vi "HP Loop.vi"(8 "error in (no error)":errorcluster, 11 "ValveControlModule in":refnum<class "DigitalControlModule.lvclass">) -> (0 "error out":errorcluster, 3 "ValveControlModule out":refnum<class "DigitalControlModule.lvclass">)   [LabVIEW 2023, in "VolatusControl.lvlib" / "DigitalControlModule.lvclass"]
uses:
  DigitalControlModule.lvclass
  DigitalControlModule.lvclass/DigitalControlModule.ctl
  <vilib>/Platform/TimedLoop/XDataNode/timing_clust.ctl
  <vilib>/Platform/TimedLoop/XDataNode/nitl_modes.ctl
  <vilib>/Platform/TimedLoop/XDataNode/wakeup.ctl
  Volatus/Module/Module.lvclass
  Volatus/Module/Module.lvclass/Module.ctl
  messages/CmdDigital/Class/Msg.lvclass
  messages/CmdDigital/Class/Msg.lvclass/Msg.ctl
  Volatus/MessageQ/MessageQ.lvclass/MessageQ.ctl
  messages/CmdDigital/Data.ctl
  messages/CmdDigitalMultiple/Data.ctl
  messages/CmdAnalog/Class/Msg.lvclass
  messages/CmdAnalog/Class/Msg.lvclass/Msg.ctl
  messages/CmdAnalog/Data.ctl
  Volatus/Module/Self Q.vi
  Volatus/MessageQ/Send.vi
  Volatus/Module/Report Event.vi
  lv-vecto/Vecto/Bool to String.vi
  lv-vecto/Vecto/Group DBL/Group DBL.lvclass
  <vilib>/Utility/error.llb/Error Cluster From Error Code.vi
  Volatus/VolatusAPI/Report Event.vi
  <vilib>/platform/TimedLoop/XDataNode/XDataNode.xnode
  <vilib>/Platform/TimedLoop/XDataNode/XDNodeRunTimeDep.lvlib
  messages/CmdDigital/CmdDigital.lvlib
  messages/CmdDigitalMultiple/CmdDigitalMultiple.lvlib
  messages/CmdAnalog/CmdAnalog.lvlib
  lv-vecto/Vecto/Group/Group.lvclass
  C:/dev/volatus/mts-volatus-super/libs/lv-volatus/Volatus/Module/Module.lvclass
  C:/dev/volatus/mts-volatus-super/libs/lv-volatus/VolatusControl/DigitalControlModule/DigitalControlModule.lvclass
  messages/CmdDigitalMultiple/Class/Msg.lvclass
  C:/dev/volatus/mts-volatus-super/libs/lv-volatus/messages/CmdDigital/Class/Msg.lvclass
  C:/dev/volatus/mts-volatus-super/libs/lv-protoc/LV-Proto/Message/Message.lvclass
  C:/dev/volatus/mts-volatus-super/libs/lv-volatus/messages/CmdDigitalMultiple/Class/Msg.lvclass
  C:/dev/volatus/mts-volatus-super/libs/lv-volatus/messages/CmdAnalog/Class/Msg.lvclass
  C:/dev/volatus/mts-volatus-super/libs/lv-vecto/Vecto/Group/Group.lvclass
  C:/dev/volatus/mts-volatus-super/libs/lv-vecto/Vecto/Group DBL/Group DBL.lvclass
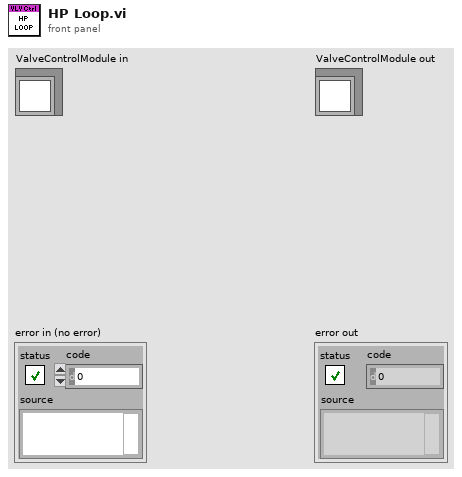
[diagram p1: front panel]
types:
  T1 = typedef "XDNodeRunTimeDep.lvlib/timing_clust.ctl" = cluster{"Expected End [f-1]":u64, "Actual End [f-1]":u64, "Finished Late? [f-1]":bool, "Expected End [i-1]":u64, "Actual End [i-1]":u64, "Finished Late? [i-1]":bool, "Expected Start [i]":u64, "Actual Start [i]":u64, "Expected Start [f]":u64, "Actual Start [f]":u64, "Source Name":string, "Structure Name":string, "Period":i64, "Deadline":i64, "Offset":i64, "Start":i64, "Priority":i32, "Timeout":i32, "Mode":T2, "Wakeup Reason":T3, "Error":errorcluster, "Source Type":string, "Secondary Source Type":string, "Global End Time":u64, "Global Start Time":u64, "Frame Duration":u64, "Iteration Duration":u64, "Assigned CPU":i32, "I/O Scan Engine Mode":u32}
  T2 = typedef "XDNodeRunTimeDep.lvlib/nitl_modes.ctl" = enum32{"No Change", "Process missed periods, maintain original phase", "Discard missed periods, maintain original phase", "Process missed periods, ignore original phase", "Discard missed periods, ignore original phase"}
  T3 = typedef "XDNodeRunTimeDep.lvlib/wakeup.ctl" = enum32{"Normal", "Aborted", "Asynchronous wakeup", "Timing source error", "Timed loop error", "Timeout"}
  T4 = enum32{"Invalid", "Standard", "Closed", "Hidden", "Minimized", "Maximized"}
  T5 = typedef "CmdDigital.lvlib/Data.ctl" = cluster{"channel":string, "value":bool}
  T6 = typedef "CmdDigitalMultiple.lvlib/Data.ctl" = cluster{"values":T5[]}
  T7 = typedef "CmdAnalog.lvlib/Data.ctl" = cluster{"channel":string, "value":dbl}
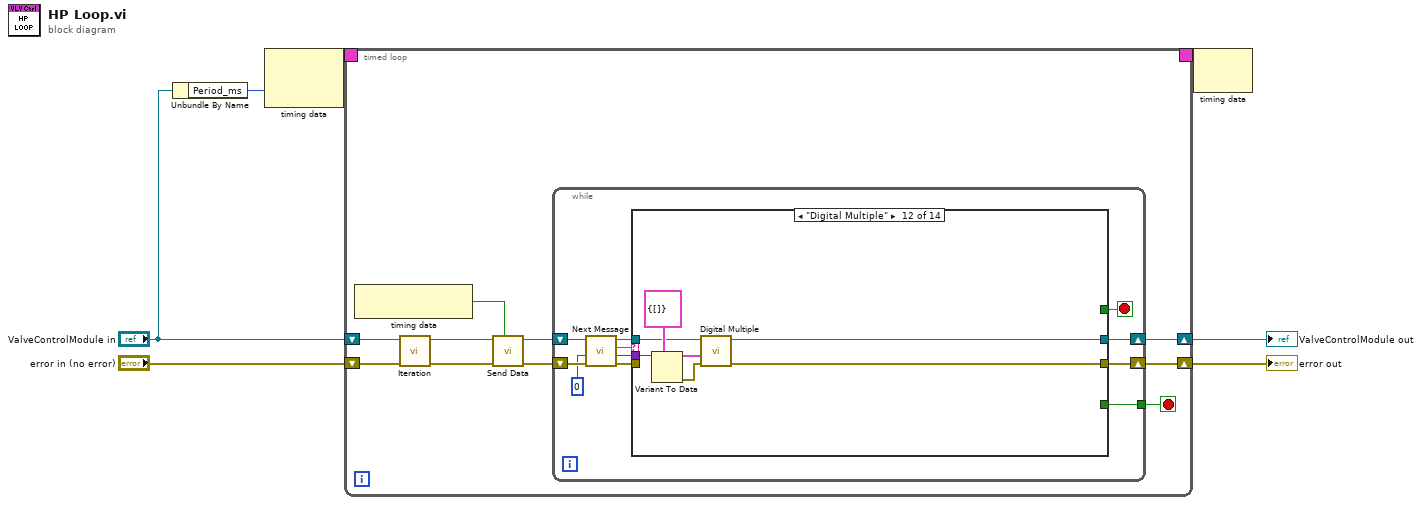
[diagram p0: block diagram]
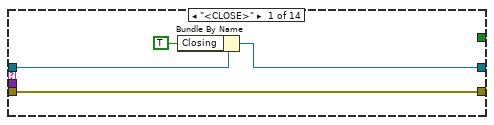
[diagram p2: hidden frame]
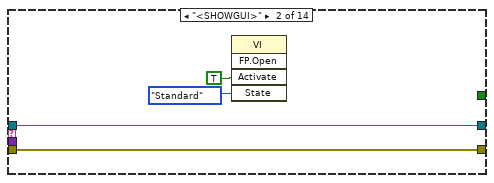
[diagram p3: hidden frame]
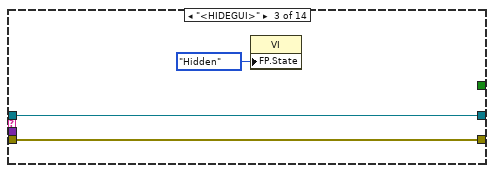
[diagram p4: hidden frame]
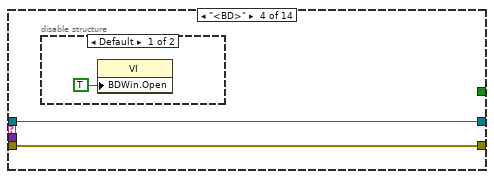
[diagram p5: hidden frame]
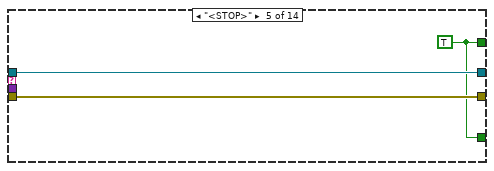
[diagram p7: hidden frame]
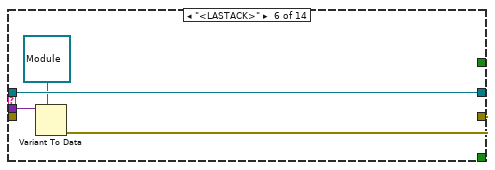
[diagram p8: hidden frame]
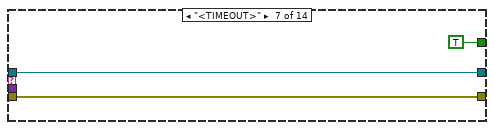
[diagram p9: hidden frame]
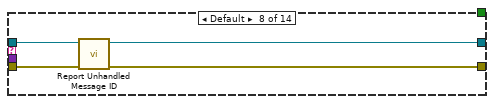
[diagram p10: hidden frame]
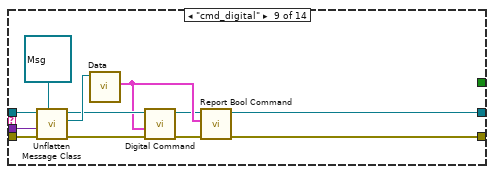
[diagram p11: hidden frame]
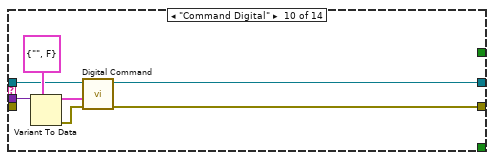
[diagram p12: hidden frame]
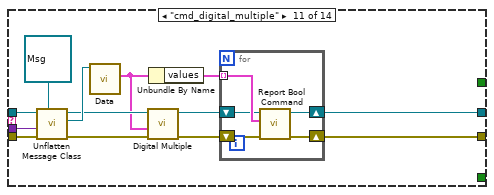
[diagram p13: hidden frame]
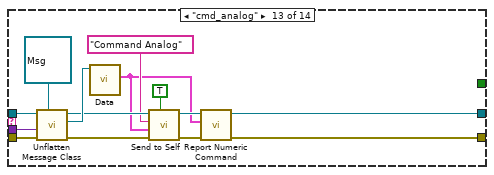
[diagram p14: hidden frame]
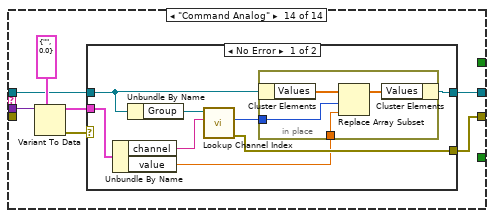
[diagram p15: hidden frame]
diagram:
  n1 = Unbundle By Name("ValveControlModule in") -> ("Period_ms"=w1:i64)
  n2 = node-c288(w1) -> (w7:T1)  [unwired: 1 in]
  n3 = timed-loop {
    shift-right: [w17] -> w4
    shift-left: "ValveControlModule in" -> [w12]
    shift-right: [w16] -> w3
    shift-left: "error in (no error)" -> [w11]
    timing: w7 -> [_]
    timing-out: [_] -> w6
    stop <- w15 stop-if-true
    n4 = node-c288() -> (w8:bool)  [unwired: 1 in]
    n5 = call "Iteration.vi"("error in (no error)"=w11, "ValveControlModule in"=w12) -> ("error out"=w13:errorcluster, "ValveControlModule out"=w14:refnum<class "DigitalControlModule.lvclass">)  [unwired: 8 in]
    n6 = call "Send Data.vi"("Finished Late"=w8, "error in (no error)"=w13, "ValveControlModule in"=w14) -> ("error out"=w10:errorcluster, "ValveControlModule out"=w9:refnum<class "DigitalControlModule.lvclass">)  [unwired: 7 in]
    n7 = while {
      tunnel: [w25] -> w15
      shift-right: [w26] -> w16
      shift-left: w10 -> [w23]
      shift-right: [w27] -> w17
      shift-left: w9 -> [w22]
      stop <- w20 stop-if-true
      n8 = call "Next Message.vi"("error in (no error)"=w23, "Timeout ms (-1)"=0, "Module in"=w22) -> ("error out"=w30:errorcluster, "Data"=w24:variant, "ID"=w29:string, "Module out"=w28:refnum<class "DigitalControlModule.lvclass">)  [unwired: 5 in]
      n9 = case shown="\"Digital Multiple\"" w29 {
        tunnel: w30 -> [w34 w37 w40 w42 w46 _ w53 w58 w69 _ w89 _ w115 _]
        tunnel: w28 -> [w33 w38 w41 w43 w47 w51 w54 w56 w70 w75 w90 w100 w116 w119]
        tunnel: [w32 w38 w41 w43 w47 w51 w54 w55 w64 w72 w84 w97 w104 w117] -> w27
        tunnel: [w34 w37 w40 w42 w46 w48 w53 w57 w65 w73 w85 w98 w106 w118] -> w26
        tunnel: [_ _ _ _ w45 _ _ _ _ _ _ _ _ _] -> w25
        tunnel: w24 -> [_ _ _ _ _ w50 _ _ w68 w77 w88 w102 w114 w123]
        tunnel: [_ _ _ _ w45 _ TRUE _ _ _ _ _ _ _] -> w20
        frame "<CLOSE>" {
          n10 = Bundle By Name(cluster=w33, "Closing"=TRUE) -> (w32:refnum<class "DigitalControlModule.lvclass">)
        }
        frame "<SHOWGUI>" {
          n11 = invoke class="VI" method="FP.Open"("Activate"=TRUE ("Activate?"), "State"=T4."Standard") -> ()  [unwired: 3 in, 5 out]
        }
        frame "<HIDEGUI>" {
          n12 = property class="VI"("FP.State"=T4."Hidden" ("Front Panel Window:State")) -> ()  [unwired: 2 in, 2 out]
        }
        frame "<BD>" {
          n13 = disable-structure shown="Default" {
            frame condition #0 (active) {
              n14 = property class="VI"("BDWin.Open"=TRUE ("Block Diagram Window:Open")) -> ()  [unwired: 2 in, 2 out]
            }
            frame condition #1 {
            }
          }
        }
        frame "<STOP>" {
          w45 = TRUE
        }
        frame "<LASTACK>" {
          n15 = Variant To Data(type=refnum<class "Module.lvclass"> refnum ("Volatus:Module"), Variant=w50) -> (error out=w48:errorcluster)  [unwired: 1 in, 1 out]
        }
        frame "<TIMEOUT>" {
        }
        frame Default {
          n16 = call "Report Unhandled Message ID.vi"("error in (no error)"=w58, "Module in"=w56) -> ("error out"=w57:errorcluster, "Module out"=w55:refnum<class "DigitalControlModule.lvclass">)  [unwired: 8 in]
        }
        frame "cmd_digital" {
          n17 = call "Unflatten Message Class.vi"("Message Type"=refnum<class "Msg.lvclass"> refnum ("CmdDigital.lvlib:Msg.lvclass"), "error in (no error)"=w69, "Data"=w68, "Module in"=w70) -> ("error out"=w62:errorcluster, "Message"=w66:refnum<class "Msg.lvclass">, "Module out"=w63:refnum<class "DigitalControlModule.lvclass">)  [unwired: 4 in, 1 out]
          n18 = call "Data.vi"("PB Msg Template in"=w66) -> ("Data"=w61:T5)  [unwired: 8 in, 2 out]
          n19 = call "Digital Command.vi"("error in (no error)"=w62, "CmdDigital"=w61, "ValveControlModule in"=w63) -> ("error out"=w59:errorcluster, "ValveControlModule out"=w60:refnum<class "DigitalControlModule.lvclass">)  [unwired: 7 in]
          n20 = call "Report Bool Command.vi"("error in (no error)"=w59, "Command"=w61, "Module in"=w60) -> ("error out"=w65:errorcluster, "Module out"=w64:refnum<class "DigitalControlModule.lvclass">)  [unwired: 7 in]
        }
        frame "Command Digital" {
          n21 = Variant To Data(type=T5 {"channel"="", "value"=FALSE} ("CmdDigital"), Variant=w77) -> (data=w71:T5, error out=w74:errorcluster)  [unwired: 1 in]
          n22 = call "Digital Command.vi"("error in (no error)"=w74, "CmdDigital"=w71, "ValveControlModule in"=w75) -> ("error out"=w73:errorcluster, "ValveControlModule out"=w72:refnum<class "DigitalControlModule.lvclass">)  [unwired: 7 in]
        }
        frame "cmd_digital_multiple" {
          n23 = call "Unflatten Message Class.vi"("Message Type"=refnum<class "Msg.lvclass"> refnum ("CmdDigitalMultiple.lvlib:Msg.lvclass"), "error in (no error)"=w89, "Data"=w88, "Module in"=w90) -> ("error out"=w82:errorcluster, "Message"=w86:refnum<class "Msg.lvclass">, "Module out"=w83:refnum<class "DigitalControlModule.lvclass">)  [unwired: 4 in, 1 out]
          n24 = call "Data.vi"("PB Msg Template in"=w86) -> ("Data"=w81:T6)  [unwired: 8 in, 2 out]
          n25 = call "Digital Multiple.vi"("error in (no error)"=w82, "Data"=w81, "ValveControlModule in"=w83) -> ("error out"=w78:errorcluster, "ValveControlModule out"=w79:refnum<class "DigitalControlModule.lvclass">)  [unwired: 7 in]
          n26 = Unbundle By Name(w81) -> ("values"=w80:T5[])
          n27 = for {
            tunnel: w80 -> [w93] mode=indexing
            shift-right: [w94] -> w84
            shift-left: w79 -> [w92]
            shift-right: [w95] -> w85
            shift-left: w78 -> [w91]
            n28 = call "Report Bool Command.vi"("error in (no error)"=w91, "Command"=w93, "Module in"=w92) -> ("error out"=w95:errorcluster, "Module out"=w94:refnum<class "DigitalControlModule.lvclass">)  [unwired: 7 in]
          }
        }
        frame "Digital Multiple" {
          n29 = Variant To Data(type=T6 {"values"=[]} ("CmdDigitalMultiple"), Variant=w102) -> (data=w99:T6, error out=w96:errorcluster)  [unwired: 1 in]
          n30 = call "Digital Multiple.vi"("error in (no error)"=w96, "Data"=w99, "ValveControlModule in"=w100) -> ("error out"=w98:errorcluster, "ValveControlModule out"=w97:refnum<class "DigitalControlModule.lvclass">)  [unwired: 7 in]
        }
        frame "cmd_analog" {
          n31 = call "Unflatten Message Class.vi"("Message Type"=refnum<class "Msg.lvclass"> refnum ("CmdAnalog.lvlib:Msg.lvclass"), "error in (no error)"=w115, "Data"=w114, "Module in"=w116) -> ("error out"=w110:errorcluster, "Message"=w112:refnum<class "Msg.lvclass">, "Module out"=w111:refnum<class "DigitalControlModule.lvclass">)  [unwired: 4 in, 1 out]
          n32 = call "Data.vi"("PB Msg Template in"=w112) -> ("Data"=w103:T7)  [unwired: 8 in, 2 out]
          n33 = call "Send to Self.vi"("High Priority (F)"=TRUE, "error in (no error)"=w110, "Data"=w103, "Message ID"="Command Analog", "Module in"=w111) -> ("error out"=w107:errorcluster, "Module out"=w105:refnum<class "DigitalControlModule.lvclass">)  [unwired: 5 in]
          n34 = call "Report Numeric Command.vi"("error in (no error)"=w107, "Command"=w103, "Module in"=w105) -> ("error out"=w106:errorcluster, "Module out"=w104:refnum<class "DigitalControlModule.lvclass">)  [unwired: 7 in]
        }
        frame "Command Analog" {
          n35 = Variant To Data(type=T7 {"channel"="", "value"=0.0} ("CmdAnalog"), Variant=w123) -> (data=w120:T7, error out=w121:errorcluster)  [unwired: 1 in]
          n36 = case shown="No Error" w121 {
            selector: w121 -> [_ w137]
            tunnel: w120 -> [w130 _]
            tunnel: w119 -> [w127 w136]
            tunnel: [w131 w137] -> w118
            tunnel: [w124 w136] -> w117
            frame No Error {
              n37 = Unbundle By Name(w130) -> ("channel"=w128:string, "value"=w125:dbl)
              n38 = Unbundle By Name(w127) -> ("Group"=w129:refnum<class "Group DBL.lvclass">)
              n39 = call "Lookup Channel Index.vi"("Channel Name"=w128, "Group in"=w129) -> ("error out"=w131:errorcluster, "Index"=w126:i32)  [unwired: 7 in, 1 out]
              n40 = in-place {
                in-place-border: w126 -> [w134]
                in-place-border: w125 -> [w133]
                n41 = in-place-cluster #1(w127) -> ("Values"=w135:dbl[])
                n42 = Replace Array Subset(array=w135, new element=w133, index=w134) -> (w132:dbl[])
                n43 = in-place-cluster #1("Values"=w132) -> (w124:refnum<class "DigitalControlModule.lvclass">)
              }
            }
            frame Error {
            }
          }
        }
      }
    }
  }
  "error out" <- w3
  "ValveControlModule out" <- w4
  n44 = node-c288(w6) -> ()  [unwired: 1 out]
